vi "read formatted default value.vi"(10 "# of Digits":u8=5, 11 "channel":refnum<class "TBM channel.lvclass">) -> (2 "Formatted Default":string, 3 "channel out":refnum<class "TBM channel.lvclass">)   [LabVIEW 2014, in "control module editor.lvclass"]
uses:
  control module editor.lvclass
  <vilib>/NI/Tag Bus Module Framework/channel/TBM channel.lvclass
  <vilib>/NI/Tag Bus/tag/tag descriptor.lvclass/tag descriptor.ctl
  <vilib>/NI/Tag Bus/tag/tag descriptor.lvclass
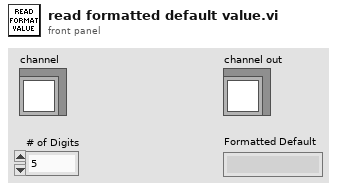
[diagram p1: front panel]
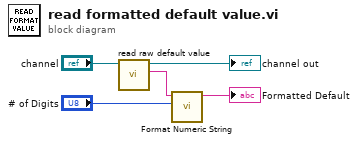
[diagram p0: block diagram]
diagram:
  n1 = call <vilib>:"read raw default value.vi"("system tag in"="channel") -> ("raw default"=w3:string, "system tag out"=→"channel out":refnum<class "TBM channel.lvclass">)  [unwired: 8 in, 1 out]
  n2 = call "Format Numeric String.vi"("digits"="# of Digits", "default value string"=w3) -> ("formatted default value string"=→"Formatted Default":string)  [unwired: 9 in]
